vi "Obtain Request Events.vi"(8 "error in":errorcluster, 10 "Create New? (F)":bool) -> (0 "error out":errorcluster, 2 "Launcher Request Events":T1)   [LabVIEW 2026, in "Launcher.lvlib"]
doc: "This VI Obtains/Creates the Requests events that will be used for other modules to communicate with the module that owns this VI. These Requests events will be accessed only via Public API methods for this module.\n\n<b>NOTE</b>: The contents of this VI are automatically generated and modified by the <b>Tools > DQMH Consortium > DQMH</b> utilities. Consider using those utilities instead of making your own modifications to this VI.\n_____\nBased on DQMH Dev Tools: Project Template 7.1.2.1547."
uses:
  Launcher.lvlib
  Request Events--cluster.ctl
  Stop Argument--cluster.ctl
  Show Panel Argument--cluster.ctl
  Hide Panel Argument--cluster.ctl
  Get Module Execution Status Argument--cluster.ctl
  Show Diagram Argument--cluster.ctl
  Set Captures Folder Argument--cluster.ctl
  Set Capture Detection Loop Timeout Argument--cluster.ctl
  Trigger Capture Detection Loop Argument--cluster.ctl
  Trigger Capture Detection Loop (Reply Payload)--cluster.ctl
  Set Application Mode Argument--cluster.ctl
  Mode.ctl
  Application Mode Argument--cluster.ctl
  Set Run ID to Replay Argument--cluster.ctl
  Set Replay Run ID Argument--cluster.ctl
panel:
  # "NOTE: The contents of this VI are automatically generated and modified by the Tools > DQMH Consortium > DQMH utilities. Consider using those utilities instead of making your own modifications to this VI."
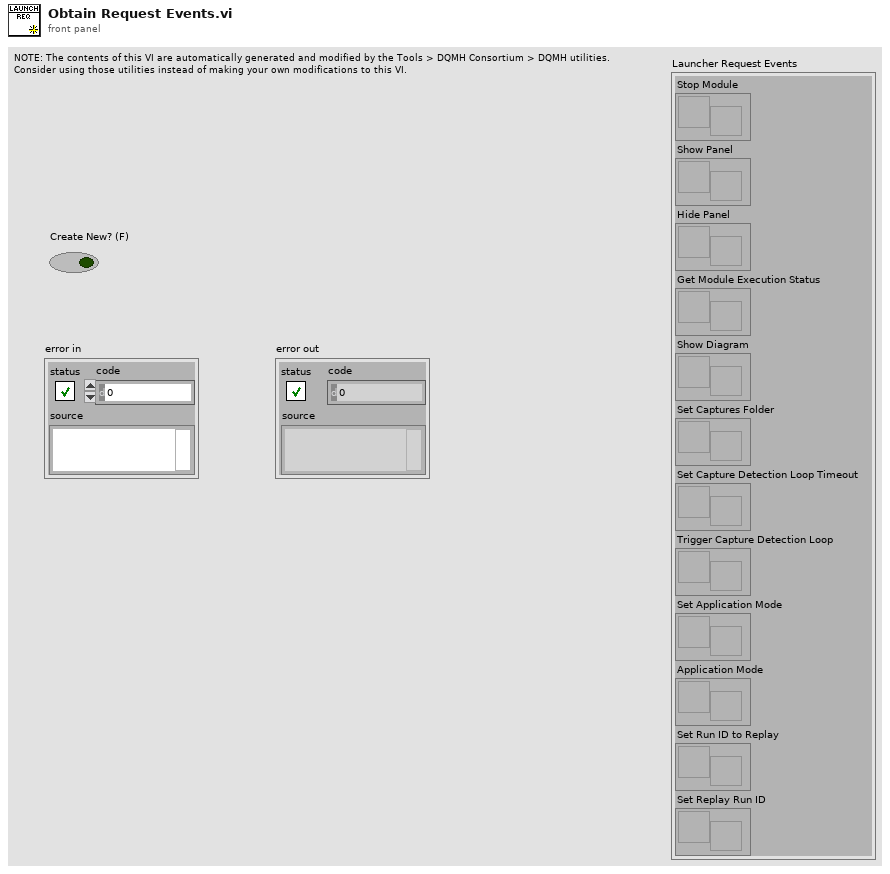
[diagram p1: front panel]
types:
  T1 = typedef "Launcher.lvlib/Request Events--cluster.ctl" = cluster{"Stop Module":refnum<user-event>, "Show Panel":refnum<user-event>, "Hide Panel":refnum<user-event>, "Get Module Execution Status":refnum<user-event>, "Show Diagram":refnum<user-event>, "Set Captures Folder":refnum<user-event>, "Set Capture Detection Loop Timeout":refnum<user-event>, "Trigger Capture Detection Loop":refnum<user-event>, "Set Application Mode":refnum<user-event>, "Application Mode":refnum<user-event>, "Set Run ID to Replay":refnum<user-event>, "Set Replay Run ID":refnum<user-event>}
  T2 = typedef "Launcher.lvlib/Set Replay Run ID Argument--cluster.ctl" = cluster{"Replay Run ID":string}
  T3 = typedef "Launcher.lvlib/Set Run ID to Replay Argument--cluster.ctl" = cluster{"Run ID":string}
  T4 = typedef "Launcher.lvlib/Application Mode Argument--cluster.ctl" = cluster{"Mode":T5}
  T5 = typedef "Mode.ctl" = enum16{"Record", "Record and Replay"}
  T6 = typedef "Launcher.lvlib/Set Application Mode Argument--cluster.ctl" = cluster{"Mode":T5}
  T7 = typedef "Launcher.lvlib/Trigger Capture Detection Loop Argument--cluster.ctl" = cluster{"Capture Detection Loop Timeout":i32, "Wait Notifier":refnum<notifier>, "wait for reply":bool}
  T8 = typedef "Launcher.lvlib/Set Capture Detection Loop Timeout Argument--cluster.ctl" = cluster{"Timeout":i32}
  T9 = typedef "Launcher.lvlib/Set Captures Folder Argument--cluster.ctl" = cluster{"Captures":path}
  T10 = typedef "Launcher.lvlib/Hide Panel Argument--cluster.ctl" = cluster{"Hide Panel?":bool}
  T11 = typedef "Launcher.lvlib/Show Panel Argument--cluster.ctl" = cluster{"Show Panel?":bool}
  T12 = typedef "Launcher.lvlib/Show Diagram Argument--cluster.ctl" = cluster{"Debug?":bool}
  T13 = typedef "Launcher.lvlib/Get Module Execution Status Argument--cluster.ctl" = cluster{"Running?":bool}
  T14 = typedef "Launcher.lvlib/Stop Argument--cluster.ctl" = cluster{"Origin":string, "Exit via Stop Module Req?":bool, "Wait for Module to stop?":bool}
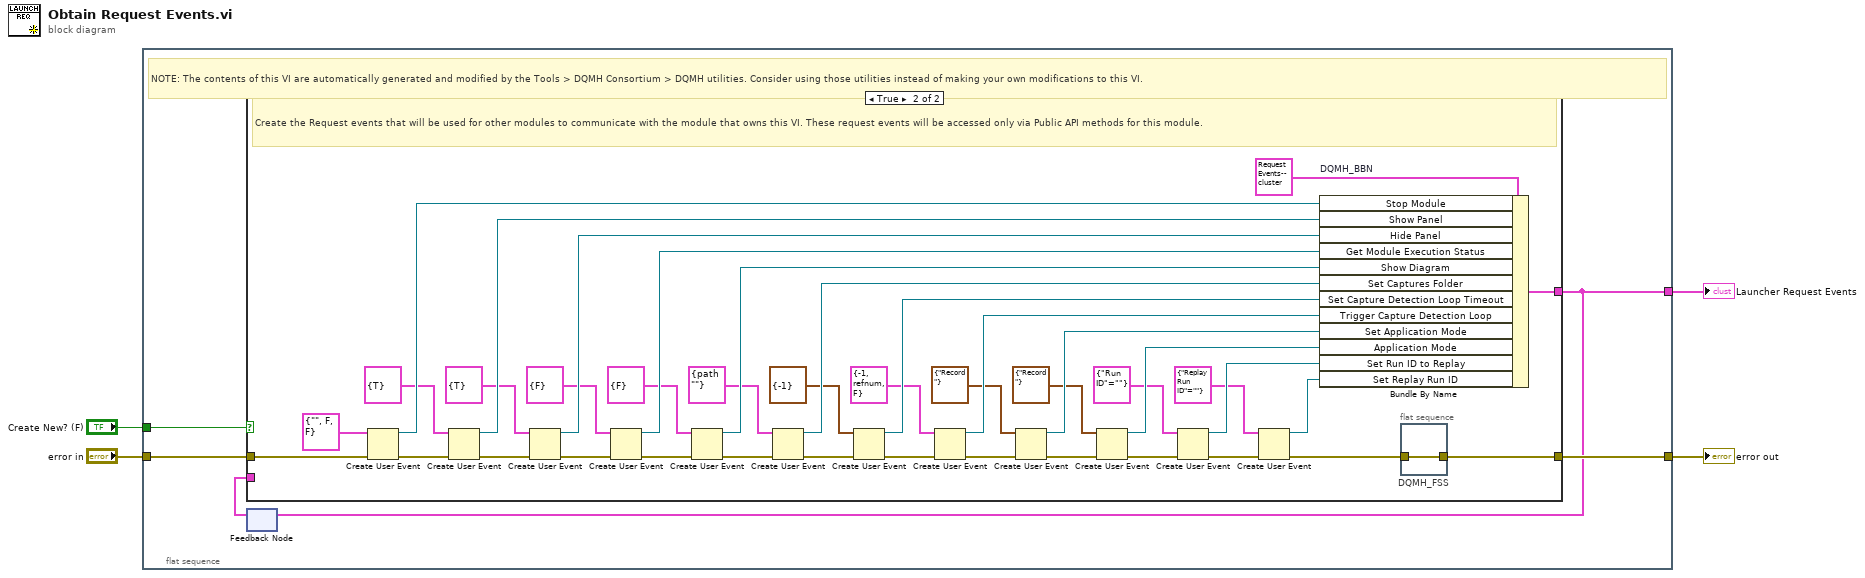
[diagram p0: block diagram]
diagram:
  n1 = flat-sequence {
    tunnel: [w9] -> w4
    tunnel: "error in" -> [w8]
    tunnel: [w6] -> w2
    tunnel: "Create New? (F)" -> [w5]
    frame #0 {
      # "NOTE: The contents of this VI are automatically generated and modified by the Tools > DQMH Consortium > DQMH utilities. Consider using those utilities instead of making your own modifications to this VI."
      n2 = feedback #1() -> (w7:T1)  [unwired: 1 in]
      n3 = case shown="True" w5 {
        tunnel: [w10 w41] -> w9
        tunnel: w8 -> [w10 w51]
        tunnel: [w11 w48] -> w6
        tunnel: w7 -> [w11 _]
        frame False {
          # "Obtain the Request events that were created in a previous call to this VI."
        }
        frame True {
          # "Create the Request events that will be used for other modules to communicate with the module that owns this VI. These request events will be accessed only via Public API methods for this module."
          n4 = Create User Event(user event datatype=T14 {"Origin"="", "Exit via Stop Module Req?"=FALSE, "Wait for Module to stop?"=FALSE} ("Stop Argument"), error in=w51) -> (user event=w49:refnum<user-event>, error out=w46:errorcluster)
          n5 = Create User Event(user event datatype=T11 {"Show Panel?"=TRUE} ("Show Panel Argument"), error in=w46) -> (user event=w45:refnum<user-event>, error out=w44:errorcluster)
          n6 = Create User Event(user event datatype=T10 {"Hide Panel?"=TRUE} ("Hide Panel Argument"), error in=w44) -> (user event=w43:refnum<user-event>, error out=w42:errorcluster)
          n7 = Create User Event(user event datatype=T13 {"Running?"=FALSE} ("Get Module Execution Status Argument"), error in=w42) -> (user event=w39:refnum<user-event>, error out=w40:errorcluster)
          n8 = Create User Event(user event datatype=T12 {"Debug?"=FALSE} ("Show Diagram Argument"), error in=w40) -> (user event=w36:refnum<user-event>, error out=w37:errorcluster)
          n9 = Create User Event(user event datatype=T9 {"Captures"=path ""} ("Set Captures Folder Argument"), error in=w37) -> (user event=w31:refnum<user-event>, error out=w32:errorcluster)
          n10 = Create User Event(user event datatype=T8 {"Timeout"=-1} ("Set Capture Detection Loop Timeout Argument"), error in=w32) -> (user event=w28:refnum<user-event>, error out=w29:errorcluster)
          n11 = Create User Event(user event datatype=T7 {"Capture Detection Loop Timeout"=-1, "Wait Notifier"=refnum, "wait for reply"=FALSE} ("Trigger Capture Detection Loop Argument"), error in=w29) -> (user event=w25:refnum<user-event>, error out=w26:errorcluster)
          n12 = Create User Event(user event datatype=T6 {"Mode"=enum."Record"} ("Set Application Mode Argument"), error in=w26) -> (user event=w22:refnum<user-event>, error out=w23:errorcluster)
          n13 = Create User Event(user event datatype=T4 {"Mode"=enum."Record"} ("Application Mode Argument"), error in=w23) -> (user event=w19:refnum<user-event>, error out=w20:errorcluster)
          n14 = Create User Event(user event datatype=T3 {"Run ID"=""} ("Set Run ID to Replay Argument"), error in=w20) -> (user event=w16:refnum<user-event>, error out=w17:errorcluster)
          n15 = Create User Event(user event datatype=T2 {"Replay Run ID"=""} ("Set Replay Run ID Argument"), error in=w17) -> (user event=w13:refnum<user-event>, error out=w14:errorcluster)
          n16 = Bundle By Name "DQMH_BBN"(cluster=T1 {"Stop Module"=refnum, "Show Panel"=refnum, "Hide Panel"=refnum, "Get Module Execution Status"=refnum, "Show Diagram"=refnum, "Set Captures Folder"=refnum, "Set Capture Detection Loop Timeout"=refnum, "Trigger Capture Detection Loop"=refnum, "Set Application Mode"=refnum, "Application Mode"=refnum, "Set Run ID to Replay"=refnum, "Set Replay Run ID"=refnum} ("output cluster"), "Stop Module"=w49, "Show Panel"=w45, "Hide Panel"=w43, "Get Module Execution Status"=w39, "Show Diagram"=w36, "Set Captures Folder"=w31, "Set Capture Detection Loop Timeout"=w28, "Trigger Capture Detection Loop"=w25, "Set Application Mode"=w22, "Application Mode"=w19, "Set Run ID to Replay"=w16, "Set Replay Run ID"=w13) -> (w48:T1)
          n17 = flat-sequence "DQMH_FSS" {
            tunnel: w14 -> [w52]
            tunnel: [w52] -> w41
            frame #0 {
            }
          }
        }
      }
      n18 = feedback-in #1(w6) -> ()
    }
  }
  "Launcher Request Events" <- w2
  "error out" <- w4
